vi "DAQmx_SyncAll.vi"(8 "error in (no error)":errorcluster, 11 "Array in":refnum<class "DAQmx.lvclass">[](array[class])) -> (0 "error out":errorcluster, 3 "Array out":refnum<class "DAQmx.lvclass">[](array[class]))   [LabVIEW 2020, in "DAQmx.lvclass"]
uses:
  DAQmx.lvclass
  DAQmx.lvclass/DAQmx.ctl
  <vilib>/DAQmx/configure/trigger.llb/DAQmx Start Trigger (Digital Edge).vi
  <resource>/objmgr/daqmx.rc
  DAQ/DAQ.lvclass
panel:
  out "Array 3":T1(array[cluster])
  out "Array 2":enum16{"MASTER", "SLAVE"}[](array[ring])
  out "Array":enum16{"MASTER", "SLAVE"}[](array[ring])
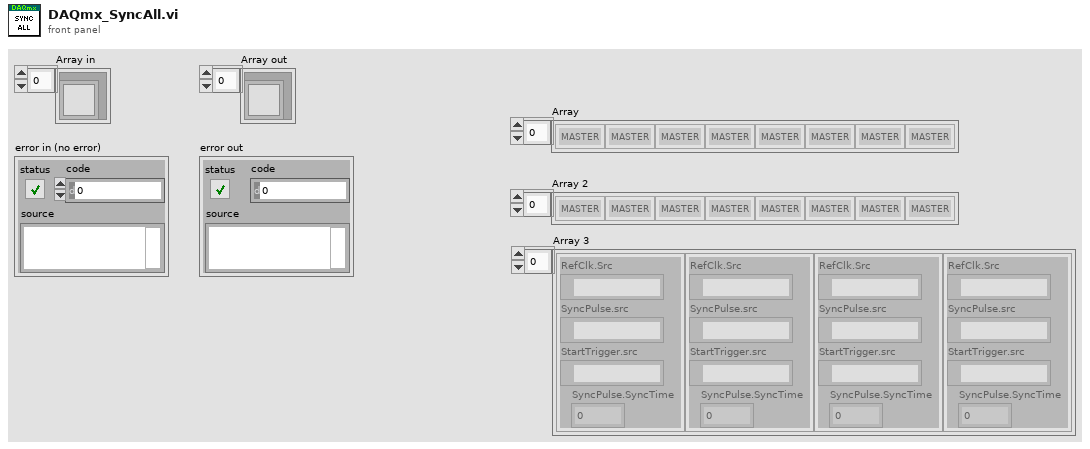
[diagram p1: front panel]
types:
  T1 = cluster{"RefClk.Src":tag, "SyncPulse.src":tag, "StartTrigger.src":tag, "SyncPulse.SyncTime":dbl}[]
  T2 = typedef "DAQmx.lvclass/DAQmx_Config.ctl" = cluster{"Buffer Size (S)":i32, "Master Slave":enum16{"MASTER", "SLAVE"}}
  T3 = cluster{"RefClk.Src":tag, "SyncPulse.src":tag, "StartTrigger.src":tag, "SyncPulse.SyncTime":dbl}
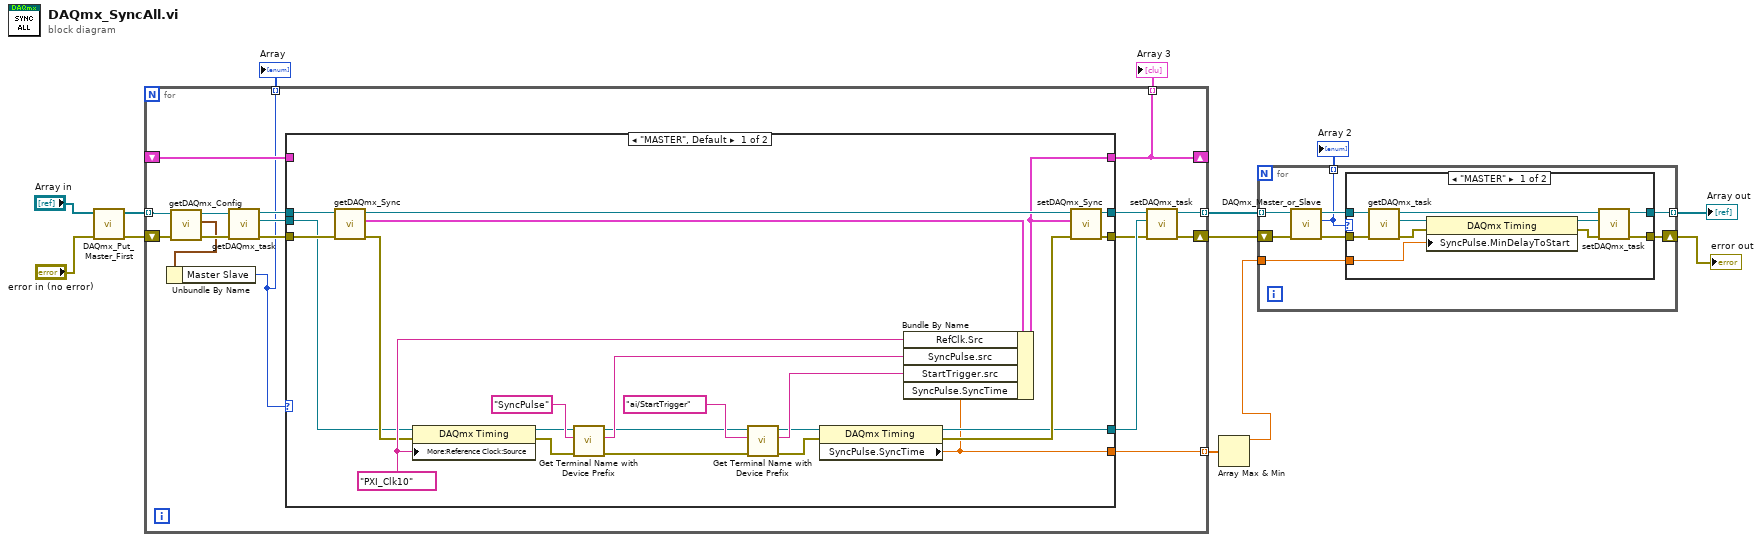
[diagram p0: block diagram]
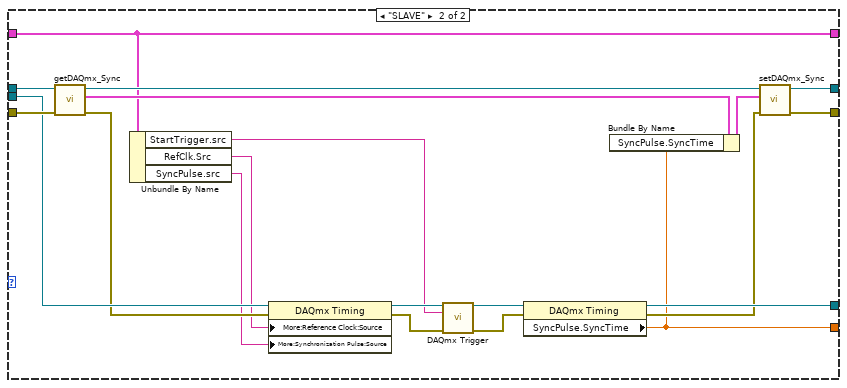
[diagram p2: hidden frame]
diagram:
  n1 = call "DAQmx_Put_Master_First.vi"("error in (no error)"="error in (no error)", "DAQmx in"="Array in") -> ("error out"=w5:errorcluster, "DAQmx out"=w6:refnum<class "DAQmx.lvclass">[])  [unwired: 8 in]
  n2 = for {
    tunnel: w6 -> [w20] mode=indexing
    shift-right: [w24] -> w10
    shift-left: w5 -> [w17]
    tunnel: [w23] -> w11 mode=indexing
    tunnel: [w22] -> w9 mode=indexing
    shift-right: [w14] -> _
    shift-left: _ -> [w21]
    tunnel: [w15] -> w4 mode=indexing
    tunnel: [w14] -> w2 mode=indexing
    n3 = call "getDAQmx_Config.vi"("error in (no error)"=w17, "DAQmx in"=w20) -> ("error out"=w18:errorcluster, "DAQmx.Config"=w16:T2, "DAQmx out"=w19:refnum<class "DAQmx.lvclass">)  [unwired: 7 in]
    n4 = Unbundle By Name(w16) -> ("Master Slave"=w15:enum16{"MASTER", "SLAVE"})
    n5 = call "getDAQmx_task.vi"("error in (no error)"=w18, "DAQmx in"=w19) -> ("error out"=w26:errorcluster, "task"=w30:refnum<k21>, "DAQmx out"=w28:refnum<class "DAQmx.lvclass">)  [unwired: 7 in]
    n6 = case shown="\"MASTER\", Default" w15 {
      tunnel: w30 -> [w35 w69]
      tunnel: [w33 w57] -> w29
      tunnel: w26 -> [w39 w70]
      tunnel: w28 -> [w42 w73]
      tunnel: [w40 w72] -> w27
      tunnel: [w36 w59] -> w25
      tunnel: [w31 w54] -> w23
      tunnel: [w32 w55] -> w14
      tunnel: w21 -> [_ w55]
      frame "MASTER", Default {
        w44 = tag "PXI_Clk10" ("RefClk.Src")
        n7 = call "getDAQmx_Sync.vi"("error in (no error)"=w39, "DAQmx in"=w42) -> ("error out"=w38:errorcluster, "Sync"=w37:T3, "DAQmx out"=w41:refnum<class "DAQmx.lvclass">)  [unwired: 7 in]
        n8 = property class="DAQmx Timing"(reference=w35, error in=w38, "More:Reference Clock:Source"=w44) -> (reference out=w51:refnum<k21>, error out=w50:errorcluster)
        n9 = call "Get Terminal Name with Device Prefix.vi"("error in (no error)"=w50, "Local Terminal Name"="SyncPulse", "task/channels in"=w51) -> ("error out"=w47:errorcluster, "Terminal Name with Device Prefix"=w49:tag, "task out"=w48:refnum<k21>)  [unwired: 6 in]
        n10 = call "Get Terminal Name with Device Prefix.vi"("error in (no error)"=w47, "Local Terminal Name"="ai/StartTrigger", "task/channels in"=w48) -> ("error out"=w43:errorcluster, "Terminal Name with Device Prefix"=w46:tag, "task out"=w45:refnum<k21>)  [unwired: 6 in]
        n11 = property class="DAQmx Timing"(reference=w45, error in=w43) -> (reference out=w33:refnum<k21>, error out=w34:errorcluster, "SyncPulse.SyncTime"=w31:dbl)
        n12 = Bundle By Name(cluster=w37, "RefClk.Src"=w44, "SyncPulse.src"=w49, "StartTrigger.src"=w46, "SyncPulse.SyncTime"=w31) -> (w32:T3)
        n13 = call "setDAQmx_Sync.vi"("error in (no error)"=w34, "Sync"=w32, "DAQmx in"=w41) -> ("error out"=w36:errorcluster, "DAQmx out"=w40:refnum<class "DAQmx.lvclass">)  [unwired: 7 in]
      }
      frame "SLAVE" {
        n14 = call "getDAQmx_Sync.vi"("error in (no error)"=w70, "DAQmx in"=w73) -> ("error out"=w68:errorcluster, "Sync"=w60:T3, "DAQmx out"=w71:refnum<class "DAQmx.lvclass">)  [unwired: 7 in]
        n15 = Unbundle By Name(w55) -> ("StartTrigger.src"=w58:tag, "RefClk.Src"=w63:tag, "SyncPulse.src"=w62:tag)
        n16 = property class="DAQmx Timing"(reference=w69, error in=w68, "More:Reference Clock:Source"=w63, "More:Synchronization Pulse:Source"=w62) -> (reference out=w66:refnum<k21>, error out=w67:errorcluster)
        n17 = call-poly <vilib>:"DAQmx Trigger.vi"("task/channels in"=w66, "source"=w58, "error in"=w67) -> ("task out"=w65:refnum<k21>, "error out"=w64:errorcluster)  [unwired: 11 in]
        n18 = property class="DAQmx Timing"(reference=w65, error in=w64) -> (reference out=w57:refnum<k21>, error out=w56:errorcluster, "SyncPulse.SyncTime"=w54:dbl)
        n19 = Bundle By Name(cluster=w60, "SyncPulse.SyncTime"=w54) -> (w61:T3)
        n20 = call "setDAQmx_Sync.vi"("error in (no error)"=w56, "Sync"=w61, "DAQmx in"=w71) -> ("error out"=w59:errorcluster, "DAQmx out"=w72:refnum<class "DAQmx.lvclass">)  [unwired: 7 in]
      }
    }
    n21 = call "setDAQmx_task.vi"("error in (no error)"=w25, "task"=w29, "DAQmx in"=w27) -> ("error out"=w24:errorcluster, "DAQmx out"=w22:refnum<class "DAQmx.lvclass">)  [unwired: 7 in]
  }
  "Array" <- w4
  "Array 3" <- w2
  n22 = Array Max & Min(array=w11) -> (max value=w1:dbl)  [unwired: 3 out]
  n23 = for {
    tunnel: w1 -> [w77]
    tunnel: w9 -> [w81] mode=indexing
    tunnel: [w76] -> w13 mode=indexing
    shift-right: [w75] -> w12
    shift-left: w10 -> [w80]
    tunnel: [w74] -> w3 mode=indexing
    n24 = call "DAQmx_Master_or_Slave.vi"("error in (no error)"=w80, "DAQmx in"=w81) -> ("error out"=w78:errorcluster, "Enum"=w74:enum16{"MASTER", "SLAVE"}, "DAQmx out"=w79:refnum<class "DAQmx.lvclass">)  [unwired: 7 in]
    n25 = case shown="\"MASTER\"" w74 {
      tunnel: w79 -> [w91 w93]
      tunnel: w78 -> [w90 w92]
      tunnel: w77 -> [w86 _]
      tunnel: [w84 w93] -> w76
      tunnel: [w83 w92] -> w75
      frame "MASTER" {
        n26 = call "getDAQmx_task.vi"("error in (no error)"=w90, "DAQmx in"=w91) -> ("error out"=w82:errorcluster, "task"=w89:refnum<k21>, "DAQmx out"=w87:refnum<class "DAQmx.lvclass">)  [unwired: 7 in]
        n27 = property class="DAQmx Timing"(reference=w89, error in=w82, "SyncPulse.MinDelayToStart"=w86) -> (reference out=w88:refnum<k21>, error out=w85:errorcluster)
        n28 = call "setDAQmx_task.vi"("error in (no error)"=w85, "task"=w88, "DAQmx in"=w87) -> ("error out"=w83:errorcluster, "DAQmx out"=w84:refnum<class "DAQmx.lvclass">)  [unwired: 7 in]
      }
      frame "SLAVE", Default {
      }
    }
  }
  "error out" <- w12
  "Array out" <- w13
  "Array 2" <- w3
